vi "Register Handler.vi"(9 "registration data":T1, 10 "indicator data in":refnum<data-value>, 11 "registry in":T2[](array[typedef])) -> (2 "indicator data out":refnum<data-value>, 3 "registry out":T2[](array[typedef]))   [LabVIEW 2018, in "GLog.lvlib" / "UI Updater.lvlib"]
uses:
  UI Updater.lvlib
  Handler Registration.ctl
  Indicator Data.ctl
  Events/Register.ctl
panel:
  # "Connector Pane"
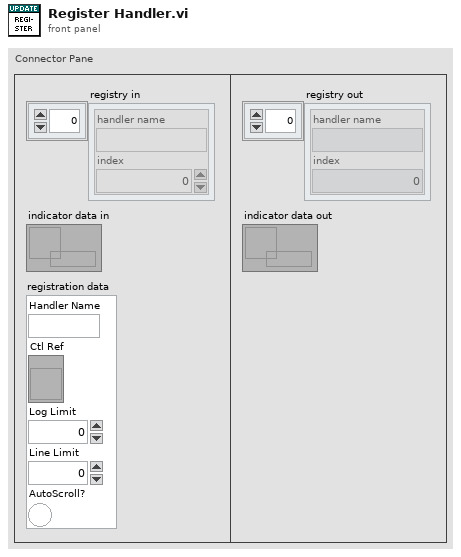
[diagram p1: front panel]
types:
  T1 = typedef "GLog.lvlib/UI Updater.lvlib/Register.ctl" = cluster{"Handler Name":string, "Ctl Ref":refnum<vi>, "Log Limit":i32, "Line Limit":i32, "AutoScroll?":bool}
  T2 = typedef "GLog.lvlib/UI Updater.lvlib/Handler Registration.ctl" = cluster{"handler name":string, "index":i32}
  T3 = typedef "GLog.lvlib/UI Updater.lvlib/Indicator Data.ctl" = cluster{"Ctl Ref":refnum<vi>, "Log Buffer":string[], "Log Limit":i32, "Line Limit":i32, "Autoscroll?":bool, "Valid?":bool, "Owning VI":refnum<vi>, "Ctl Index":i32, "Needs Write?":bool}
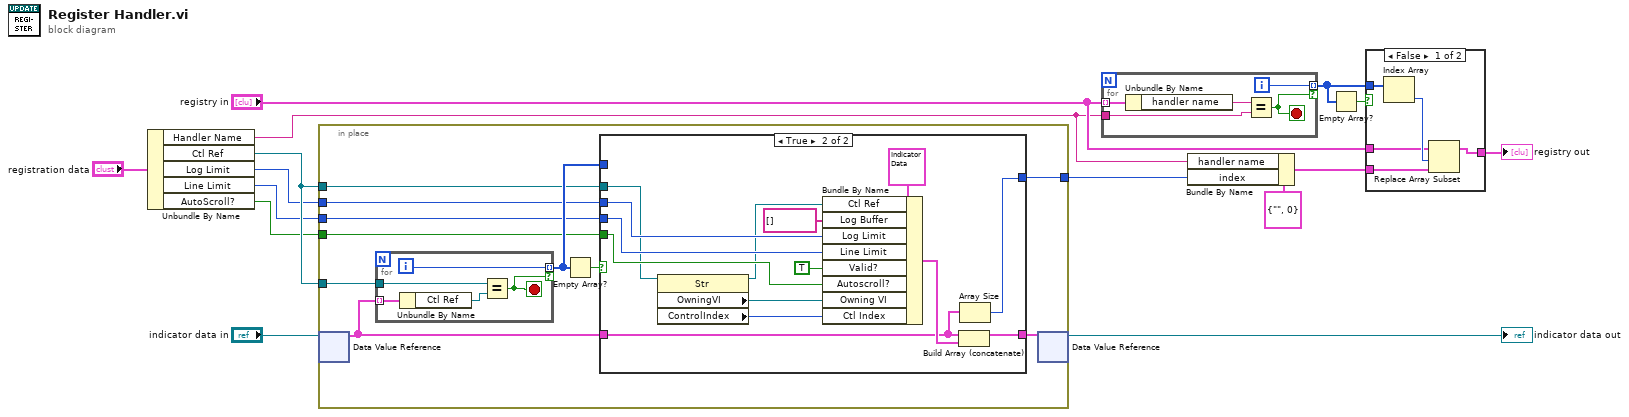
[diagram p0: block diagram]
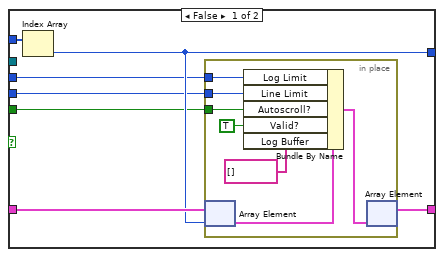
[diagram p2: hidden frame]
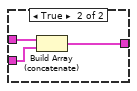
[diagram p3: hidden frame]
diagram:
  n1 = Unbundle By Name("registration data") -> ("Handler Name"=w5:string, "Ctl Ref"=w4:refnum<vi>, "Log Limit"=w3:i32, "Line Limit"=w2:i32, "AutoScroll?"=w1:bool)
  n2 = in-place {
    in-place-border: w4 -> [w25]
    in-place-border: w4 -> [w20]
    in-place-border: w3 -> [w19]
    in-place-border: w2 -> [w18]
    in-place-border: [w17] -> w14
    in-place-border: w1 -> [w16]
    n3 = in-place-dvr #1("indicator data in") -> (w21:T3[])  [unwired: 1 out]
    n4 = for {
      tunnel: w21 -> [w58] mode=indexing
      tunnel: w25 -> [w56]
      tunnel: [w55] -> w24 mode=indexing if=w54
      i -> [w55]
      stop <- w54 stop-if-true
      n5 = Unbundle By Name(w58) -> ("Ctl Ref"=w57:refnum<vi>)
      n6 = Equal?(x=w56, y=w57) -> (x = y?=w54:bool)
    }
    n7 = Empty Array?(array=w24) -> (empty?=w23:bool)
    n8 = case shown="True" w23 {
      tunnel: w24 -> [w32 _]
      tunnel: [w27 w48] -> w22
      tunnel: w21 -> [w31 w46]
      tunnel: w20 -> [_ w40]
      tunnel: w19 -> [w29 w51]
      tunnel: w18 -> [w28 w50]
      tunnel: [w30 w45] -> w17
      tunnel: w16 -> [w26 w42]
      frame False {
        n9 = Index Array(array=w32) -> (element=w30:i32)  [unwired: 1 in]
        n10 = in-place {
          in-place-border: w29 -> [w37]
          in-place-border: w28 -> [w36]
          in-place-border: w26 -> [w34]
          n11 = in-place-array #2(w31, w30) -> (w39:T3)
          n12 = Bundle By Name(cluster=w39, "Log Limit"=w37, "Line Limit"=w36, "Autoscroll?"=w34, "Valid?"=TRUE, "Log Buffer"=string[] [] ("log buffer")) -> (w35:T3)
          n13 = in-place-array #2(w35) -> (w27:T3[])  [unwired: 1 out]
        }
      }
      frame True {
        n14 = property class="Str"(reference=w40) -> (reference out=w41:refnum<vi>, "OwningVI"=w44:refnum<vi>, "ControlIndex"=w43:i32)  [unwired: 1 in, 1 out]
        n15 = Bundle By Name(cluster=T3 {"Ctl Ref"=refnum, "Log Buffer"=[], "Log Limit"=0, "Line Limit"=0, "Autoscroll?"=FALSE, "Valid?"=FALSE, "Owning VI"=refnum, "Ctl Index"=0, "Needs Write?"=FALSE}, "Ctl Ref"=w41, "Log Buffer"=string[] [] ("log buffer"), "Log Limit"=w51, "Line Limit"=w50, "Valid?"=TRUE, "Autoscroll?"=w42, "Owning VI"=w44, "Ctl Index"=w43) -> (w47:T3)
        n16 = Build Array (concatenate)(w46, w47) -> (w48:T3[])
        n17 = Array Size(array=w46) -> (size(s)=w45:i32)
      }
    }
    n18 = in-place-dvr #1(w22) -> (→"indicator data out":refnum<data-value>)  [unwired: 1 out]
  }
  n19 = for {
    tunnel: "registry in" -> [w63] mode=indexing
    tunnel: w5 -> [w62]
    tunnel: [w60] -> w10 mode=indexing if=w59
    i -> [w60]
    stop <- w59 stop-if-true
    n20 = Unbundle By Name(w63) -> ("handler name"=w61:string)
    n21 = Equal?(x=w61, y=w62) -> (x = y?=w59:bool)
  }
  n22 = Bundle By Name(cluster=T2 {"handler name"="", "index"=0} ("registration"), "handler name"=w5, "index"=w14) -> (w15:T2)
  n23 = Empty Array?(array=w10) -> (empty?=w9:bool)
  n24 = case shown="False" w9 {
    tunnel: w10 -> [w68 _]
    tunnel: "registry in" -> [w66 w71]
    tunnel: [w65 w69] -> w12
    tunnel: w15 -> [w64 w70]
    frame False {
      n25 = Index Array(array=w68) -> (element=w67:i32)  [unwired: 1 in]
      n26 = Replace Array Subset(array=w66, new element=w64, index=w67) -> (w65:T2[])
    }
    frame True {
      n27 = Build Array (concatenate)(w71, w70) -> (w69:T2[])
    }
  }
  "registry out" <- w12
